vi "sync init shared memory.vi"(7 "permissions (0664)":T1={"owner"={"read"=TRUE, "write"=TRUE, "execute"=FALSE}, "group"={"read"=TRUE, "write"=TRUE, "execute"=FALSE}, "everyone"={"read"=TRUE, "write"=TRUE, "execute"=FALSE}}, 8 "error in (no error)":errorcluster, 11 "sync shm name":string) -> (0 "error out":errorcluster, 2 "pointer to shared memory":u64, 3 "shared memory out":T2)   [LabVIEW 2014, in "Shared Memory runtime.lvclass"]
uses:
  Shared Memory runtime.lvclass
  <vilib>/NI/NI Linux RT IPC/Shared Memory/Controls/reference.ctl
  <vilib>/NI/NI Linux RT IPC/Shared Memory/Classes/Shared Memory/Shared Memory.lvclass
  <vilib>/NI/NI Linux RT IPC/Shared Memory/Controls/file mode.ctl
  <vilib>/NI/NI Linux RT IPC/Shared Memory/Linux RT IPC.Shared Memory.lvlib
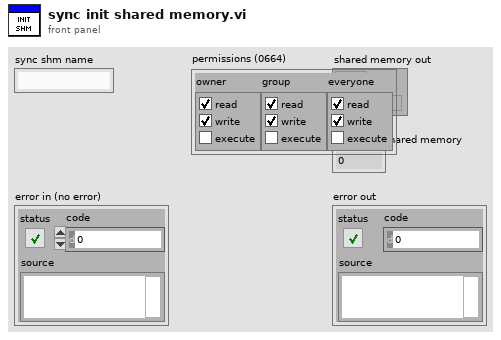
[diagram p1: front panel]
types:
  T1 = cluster{"owner":cluster{"read":bool, "write":bool, "execute":bool}, "group":cluster{"read":bool, "write":bool, "execute":bool}, "everyone":cluster{"read":bool, "write":bool, "execute":bool}}
  T2 = typedef "Linux RT IPC.Shared Memory.lvlib/reference.ctl" = refnum<data-value>
  T3 = typedef "Linux RT IPC.Shared Memory.lvlib/file mode.ctl" = enum16{"open", "create/replace"}
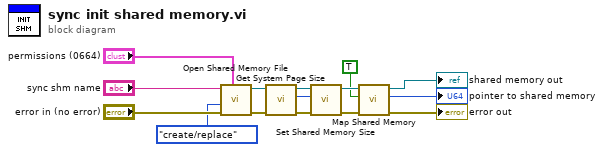
[diagram p0: block diagram]
diagram:
  n1 = call <vilib>:"Open Shared Memory File.vi"("permissions (0664)"="permissions (0664)", "error in (no error)"="error in (no error)", "file mode (open)"=file_mode."create/replace", "shared memory name"="sync shm name") -> ("error out"=w6:errorcluster, "shared memory out"=w7:T2)  [unwired: 6 in]
  n2 = call <vilib>:"Get System Page Size.vi"("error in (no error)"=w6, "shared memory in"=w7) -> ("error out"=w8:errorcluster, "page size (bytes)"=w10:u32, "shared memory out"=w9:T2)  [unwired: 7 in]
  n3 = call <vilib>:"Set Shared Memory Size.vi"("error in (no error)"=w8, "size (bytes)"=w10, "shared memory in"=w9) -> ("error out"=w12:errorcluster, "shared memory out"=w11:T2)  [unwired: 7 in]
  n4 = call <vilib>:"Map Shared Memory.vi"("error in (no error)"=w12, "close file descriptor on success? (F)"=TRUE, "shared memory in"=w11) -> ("error out"=→"error out":errorcluster, "pointer to shared memory"=→"pointer to shared memory":u64, "shared memory out"=→"shared memory out":T2)  [unwired: 6 in]
